vi "Write Transport.vi"(8 "error in":errorcluster, 10 "data in":string, 11 "transport_session":T2) -> (0 "error out":errorcluster, 2 "bytes written":u32, 3 "transport_session out":T2)   [LabVIEW 2015, in "Lengmur_socket.lvlib"]
uses:
  Lengmur_socket.lvlib
  Types/Transport Kind.ctl
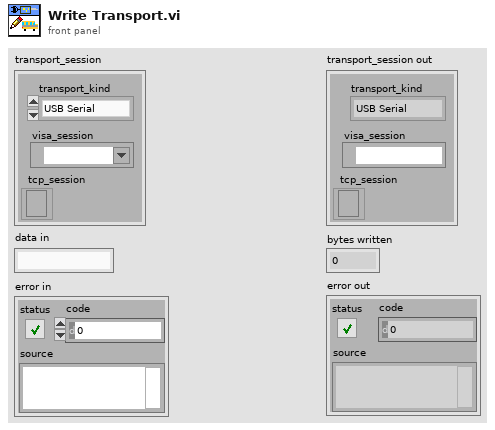
[diagram p1: front panel]
types:
  T1 = typedef "Lengmur_socket.lvlib/Transport Kind.ctl" = enum16{"USB Serial", "Ethernet TCP"}
  T2 = cluster{"transport_kind":T1, "visa_session":refnum<visa-resource-name>, "tcp_session":refnum<k5>}
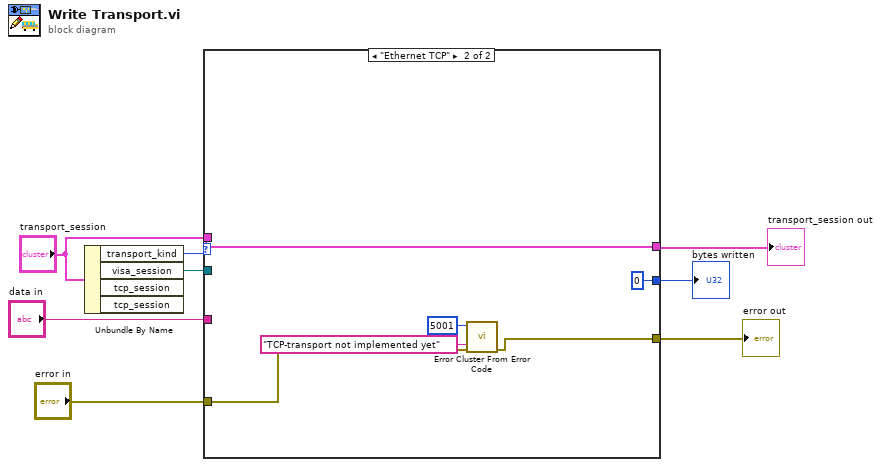
[diagram p0: block diagram]
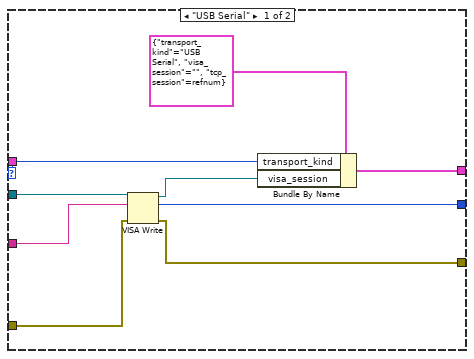
[diagram p2: hidden frame]
diagram:
  n1 = Unbundle By Name("transport_session") -> ("transport_kind"=w8:T1, "visa_session"=w5:refnum<visa-resource-name>)  [unwired: 2 out]
  n2 = case shown="\"Ethernet TCP\"" w8 {
    selector: w8 -> [w10 _]
    tunnel: "error in" -> [w17 w21]
    tunnel: "data in" -> [w16 _]
    tunnel: w5 -> [w15 _]
    tunnel: [w14 u32 0 ("return count")] -> w4
    tunnel: [w13 w20] -> w3
    tunnel: [w9 w22] -> w2
    tunnel: "transport_session" -> [_ w22]
    frame "USB Serial" {
      n3 = VISA Write(VISA resource name=w15, write buffer=w16, error in (no error)=w17) -> (VISA resource name out=w11:refnum<visa-resource-name>, return count=w14:u32, error out=w13:errorcluster)
      n4 = Bundle By Name(cluster=T2 {"transport_kind"=enum."USB Serial", "visa_session"="", "tcp_session"=refnum} ("transport_session"), "transport_kind"=w10, "visa_session"=w11) -> (w9:T2)
    }
    frame "Ethernet TCP" {
      n5 = call <vilib>:"Error Cluster From Error Code.vi"("error in (no error)"=w21, "error message (\"\")"="TCP-transport not implemented yet" ("error message (\"\")"), "error code (0)"=5001) -> ("error out"=w20:errorcluster)  [unwired: 6 in]
    }
  }
  "transport_session out" <- w2
  "bytes written" <- w4
  "error out" <- w3
